vi "Mise en forme profil EPC3000.vi"(0 "Début du profil":timestamp format="%<%H:%M:%S\n%A %d/%m/%y>T", 1 "Port COM run 1 REG":refnum<visa-resource-name> caption="Port RS232", 2 "Val T ini en entrée":dbl, 3 "Onglet_Tinit":enum32{"Définir Tinit", "Acquérir Tinit"}(tab), 4 "Config + programmes":T2 {"Prog 10 en sortie"."?" format="%.2f"; "Prog 9 en sortie"."?" format="%.2f"; "Prog 8 en sortie"."?" format="%.2f"; "Prog 7 en sortie"."?" format="%.2f"; "Prog 6 en sortie"."?" format="%.2f"; "Prog 5 en sortie"."?" format="%.2f"; "config"."value" format="%.2f"; "Prog 1 en sortie"."?" format="%.2f"; "Prog 2 en sortie"."?" format="%.2f"; "Prog 3 en sortie"."?" format="%.2f"; "Prog 4 en sortie"."?" format="%.2f"}, 5 "adresse reg":u8) -> (6 "Graphe XY":cluster{"Y":dbl[], "Y":dbl[]}[](array[cluster]), 7 "Type de fin":string, 8 "Courbes à afficher":bool[](array[boolean]), 9 "Bornes profil":T1, 10 "Listing_sortie":string)   [LabVIEW 2022 SP3]
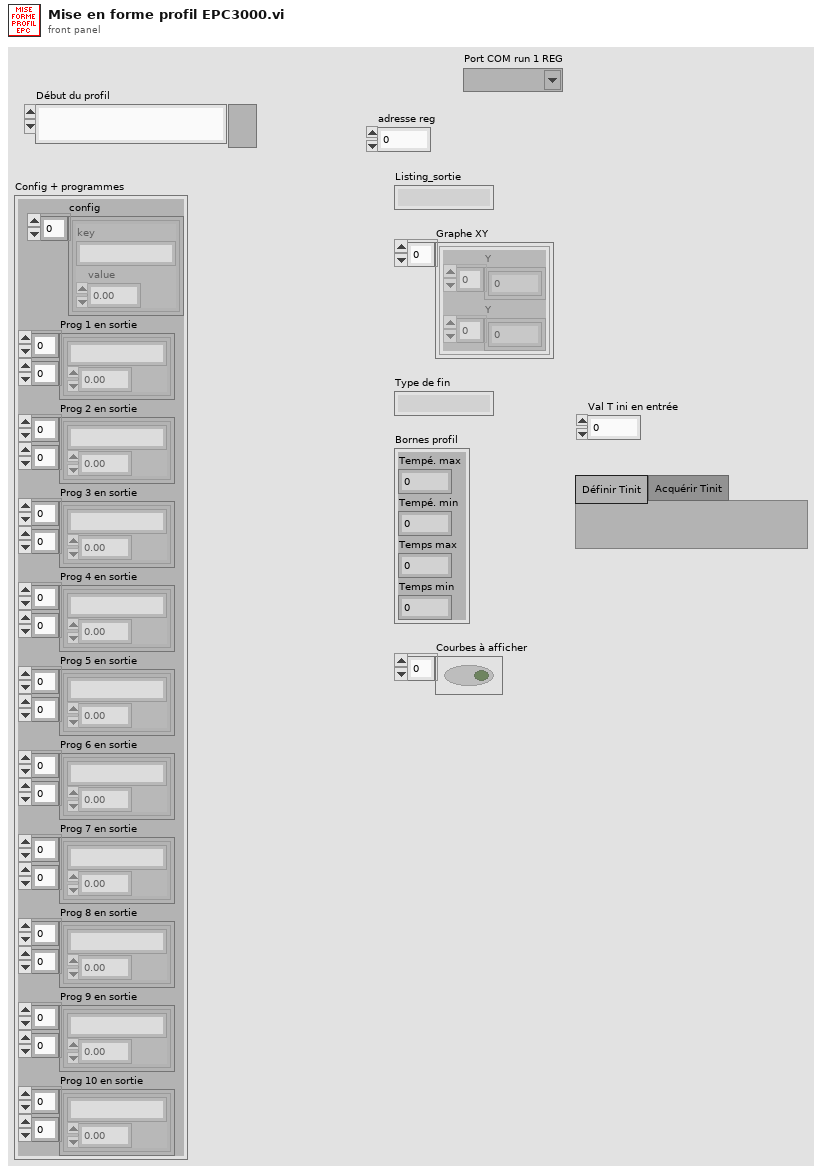
[diagram p1: front panel]
types:
  T1 = cluster{"Tempé. max":dbl, "Tempé. min":dbl, "Temps max":dbl, "Temps min":dbl}
  T2 = cluster{"config":cluster{"key":string, "value":dbl}[], "Prog 1 en sortie":cluster{string, dbl}[][], "Prog 2 en sortie":cluster{string, dbl}[][], "Prog 3 en sortie":cluster{string, dbl}[][], "Prog 4 en sortie":cluster{string, dbl}[][], "Prog 5 en sortie":cluster{string, dbl}[][], "Prog 6 en sortie":cluster{string, dbl}[][], "Prog 7 en sortie":cluster{string, dbl}[][], "Prog 8 en sortie":cluster{string, dbl}[][], "Prog 9 en sortie":cluster{string, dbl}[][], "Prog 10 en sortie":cluster{string, dbl}[][]}
  T3 = cluster{"Ev_Saut":dbl[], "Ev_Palier":dbl[], "Ev_Rampe_vitesse":dbl[], "Ev_Rampe_temps":dbl[], "Ev_Appel":dbl[], "Ev_Fin":dbl[], "T_Fin":dbl[], "T_Appel":dbl[], "T_Rampe_temps":dbl[], "T_Rampe_vitesse":dbl[], "T_Palier":dbl[], "T_Saut":dbl[], "Type de fin":string}
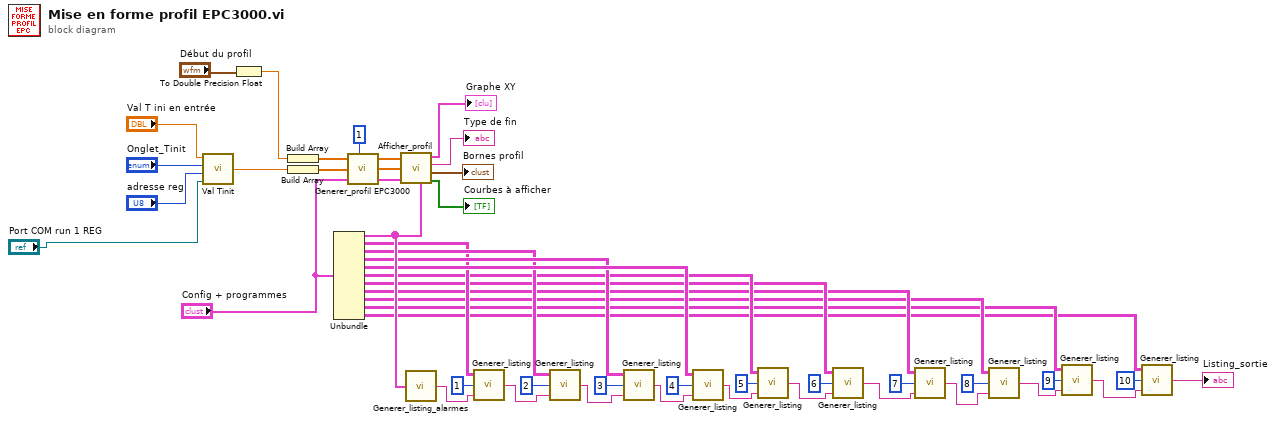
[diagram p0: block diagram]
diagram:
  n1 = call "Val Tinit.vi"("Port COM run 1 REG"="Port COM run 1 REG", "Adresse"="adresse reg", "Onglet_Tinit"="Onglet_Tinit", "Val T ini"="Val T ini en entrée") -> ("Température"=w48:dbl)
  n2 = To Double Precision Float(number="Début du profil") -> (double precision float=w44:dbl)
  n3 = Build Array(w44) -> (w25:dbl[])
  n4 = Build Array(w48) -> (w24:dbl[])
  n5 = Unbundle("Config + programmes") -> ("config"=w43:cluster{"key":string, "value":dbl}[], "Prog 1 en sortie"=w38:cluster{string, dbl}[][], "Prog 2 en sortie"=w39:cluster{string, dbl}[][], "Prog 3 en sortie"=w40:cluster{string, dbl}[][], "Prog 4 en sortie"=w41:cluster{string, dbl}[][], "Prog 5 en sortie"=w7:cluster{string, dbl}[][], "Prog 6 en sortie"=w6:cluster{string, dbl}[][], "Prog 7 en sortie"=w5:cluster{string, dbl}[][], "Prog 8 en sortie"=w4:cluster{string, dbl}[][], "Prog 9 en sortie"=w3:cluster{string, dbl}[][], "Prog 10 en sortie"=w2:cluster{string, dbl}[][])
  n6 = call "Generer_profil EPC3000.vi"("Temps (s)"=w25, "Num_Prog"=u8 1, "Températures (°C)"=w24, "Programmes et config"="Config + programmes") -> ("Temps (s)"=w26:dbl[], "Températures (°C)"=w28:dbl[], "Evennements_sortie"=w27:T3)  [unwired: 1 in]
  n7 = call "Afficher_profil.vi"("Configuration"=w43, "Temps (s)"=w26, "Températures (°C)"=w28, "Evennements_entrée"=w27) -> ("Graphe XY"=→"Graphe XY":cluster{"Y":dbl[], "Y":dbl[]}[], "Type de fin"=→"Type de fin":string, "Bornes profil"=→"Bornes profil":T1, "Courbes à afficher"=→"Courbes à afficher":bool[])
  n8 = call "Generer_listing_alarmes.vi"("Configuration"=w43) -> ("Listing alarmes"=w42:string)
  n9 = call "Generer_listing.vi"("Listing_entrée"=w42, "Numéro de programme"=u8 1, "Programme"=w38) -> ("Listing_sortie"=w31:string)
  n10 = call "Generer_listing.vi"("Listing_entrée"=w31, "Numéro de programme"=u8 2, "Programme"=w39) -> ("Listing_sortie"=w32:string)
  n11 = call "Generer_listing.vi"("Listing_entrée"=w32, "Numéro de programme"=u8 3, "Programme"=w40) -> ("Listing_sortie"=w33:string)
  n12 = call "Generer_listing.vi"("Listing_entrée"=w33, "Numéro de programme"=u8 4, "Programme"=w41) -> ("Listing_sortie"=w9:string)
  n13 = call "Generer_listing.vi"("Listing_entrée"=w9, "Numéro de programme"=u8 5, "Programme"=w7) -> ("Listing_sortie"=w19:string)
  n14 = call "Generer_listing.vi"("Listing_entrée"=w19, "Numéro de programme"=u8 6, "Programme"=w6) -> ("Listing_sortie"=w18:string)
  n15 = call "Generer_listing.vi"("Listing_entrée"=w18, "Numéro de programme"=u8 7, "Programme"=w5) -> ("Listing_sortie"=w17:string)
  n16 = call "Generer_listing.vi"("Listing_entrée"=w17, "Numéro de programme"=u8 8, "Programme"=w4) -> ("Listing_sortie"=w1:string)
  n17 = call "Generer_listing.vi"("Listing_entrée"=w1, "Numéro de programme"=u8 9, "Programme"=w3) -> ("Listing_sortie"=w10:string)
  n18 = call "Generer_listing.vi"("Listing_entrée"=w10, "Numéro de programme"=u8 10, "Programme"=w2) -> ("Listing_sortie"=→"Listing_sortie":string)
